vi "Target E.vi"(0 "x":dbl, 11 "error in":errorcluster) -> (4 "x times two":dbl, 15 "error out":errorcluster)   [LabVIEW 2026]
doc: "Returns x multiplied by two."
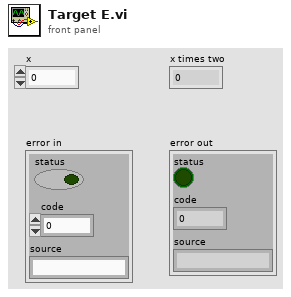
[diagram p1: front panel]
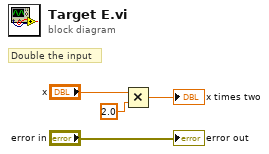
[diagram p0: block diagram]
diagram:
  # "Double the input"
  n1 = Multiply(x="x", y=2.0) -> (x*y=→"x times two":dbl)
  "error out" <- "error in"
